vi "Load_ESR.vi"(8 "Tset setting":dbl=800.0, 9 "N per point":i32=7, 10 "wait time adjustment (":dbl, 11 "wait time adjustment":dbl) -> (0 "Unaveraged data":string[][](array[string]), 1 "Array":string[][](array[string]), 2 "Data":string[][](array[string]))   [LabVIEW 2025]
uses:
  MW_resource_name.vi
panel:
  out "error out 3":errorcluster
  out "reference out":refnum<k15>
  in  "RF:Power Level (dBm)":dbl
  in  "Invert pass?":bool=TRUE
  out "Passes":i32
  in  "How many passes?":i32=3
  out "Total Points":dbl
  in  "Step Size":string=".25"
  in  "Ending Frequency":string="3100"
  in  "Starting frequency":string="2650"
  # "A gate delay Typically at 1.25 us\nwidth 300 ns"
  # "18.5 Max"
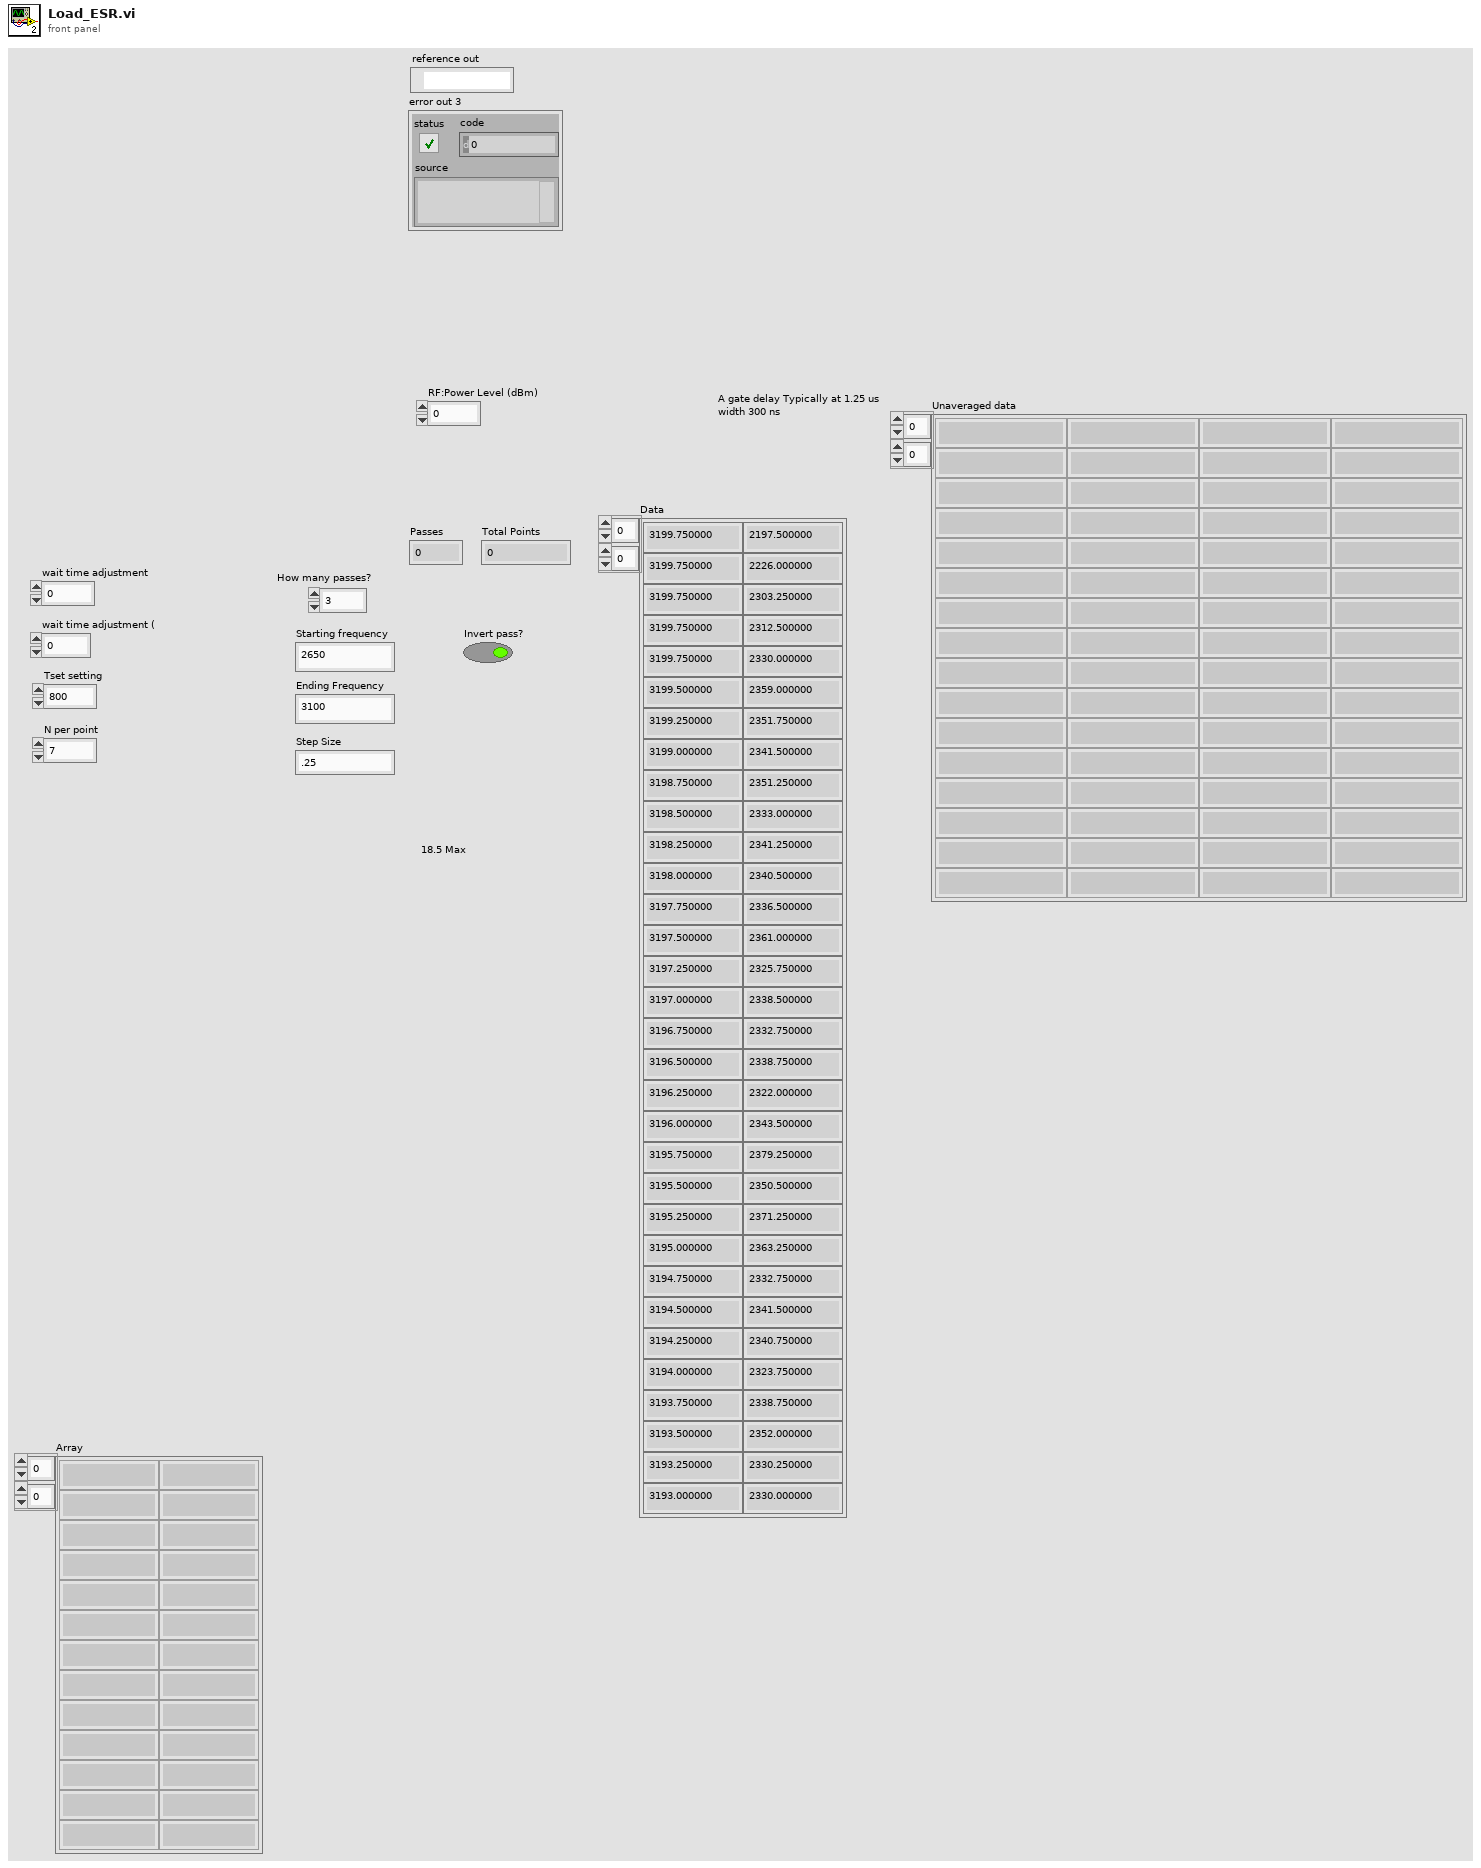
[diagram p1: front panel]
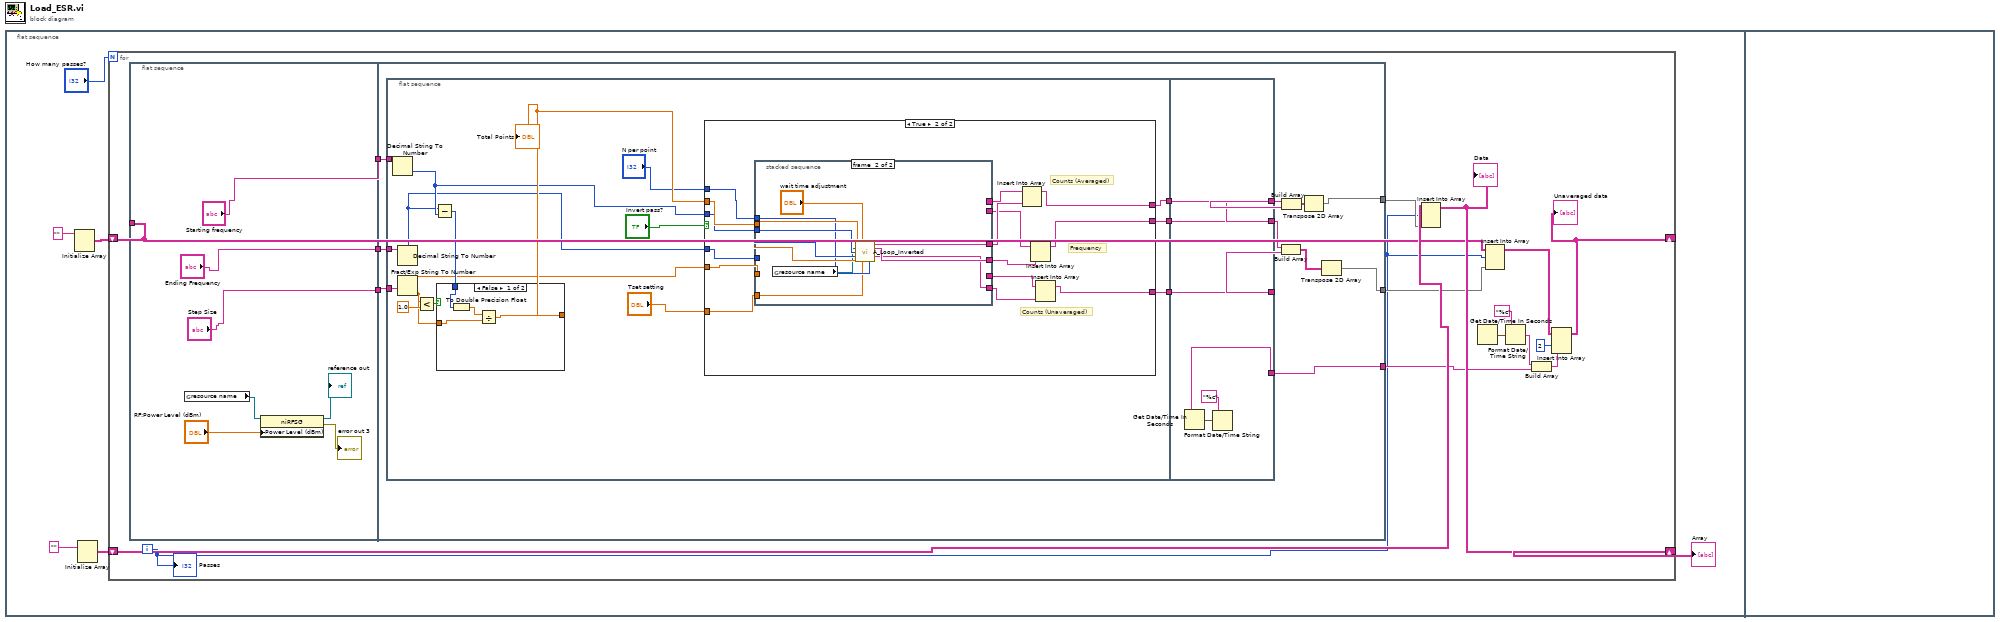
[diagram p0: block diagram]
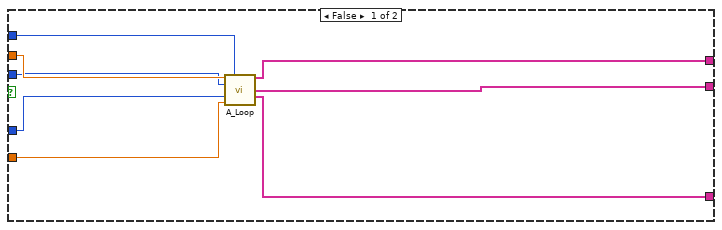
[diagram p2: hidden frame]
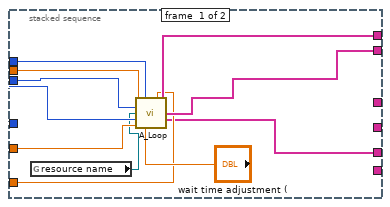
[diagram p3: hidden frame]
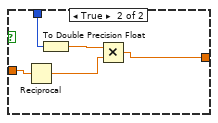
[diagram p4: hidden frame]
diagram:
  n1 = flat-sequence {
    frame #0 {
      n2 = Initialize Array("") -> (w1:string[][])  [unwired: 2 in]
      n3 = Initialize Array("") -> (w4:string[][])  [unwired: 2 in]
      n4 = for {
        N: "How many passes?" -> [_]
        shift-right: [w19] -> w3
        shift-left: w4 -> [w20]
        shift-right: [w12] -> _
        shift-left: w1 -> [w11]
        i -> [w7]
        n5 = flat-sequence {
          tunnel: ["Starting frequency"] -> w23
          tunnel: ["Ending Frequency"] -> w22
          tunnel: ["Step Size"] -> w21
          tunnel: w11 -> [_]
          tunnel: w23 -> [w44]
          tunnel: w22 -> [w43]
          tunnel: w21 -> [w42]
          tunnel: [w40] -> w9
          tunnel: [w38] -> w18
          tunnel: [w31] -> w8
          frame #0 {
            n6 = global read "MW_resource_name.vi" "resource name"() -> (w24:refnum<k15>)
            n7 = property class="niRFSG"(reference=w24, "Power Level (dBm)"="RF:Power Level (dBm)") -> (reference out=→"reference out":refnum<k15>, error out=→"error out 3":errorcluster)  [unwired: 1 in]
          }
          frame #1 {
            n8 = flat-sequence {
              tunnel: w44 -> [w60]
              tunnel: w43 -> [w59]
              tunnel: w42 -> [w57]
              tunnel: [w45] -> w34
              tunnel: [w47] -> w33
              tunnel: [w46] -> w32
              tunnel: [w118] -> w36
              tunnel: [w119] -> w37
              tunnel: [w120] -> w39
              tunnel: w34 -> [w120]
              tunnel: w33 -> [w119]
              tunnel: w32 -> [w118]
              tunnel: [w115] -> w31
              frame #0 {
                n9 = Decimal String To Number(string=w60) -> (number=w52:i32)  [unwired: 2 in, 1 out]
                n10 = Decimal String To Number(string=w59) -> (number=w51:i32)  [unwired: 2 in, 1 out]
                n11 = Fract/Exp String To Number(string=w57) -> (number=w50:dbl)  [unwired: 3 in, 1 out]
                n12 = Less?(x=w50, y=1.0) -> (x < y?=w58:bool)
                n13 = Subtract(x=w51, y=w52) -> (x-y=w55:i32)
                n14 = case shown="False" w58 {
                  tunnel: w50 -> [w107 w114]
                  tunnel: w55 -> [w109 w112]
                  tunnel: [w106 w110] -> w53
                  frame False {
                    n15 = To Double Precision Float(number=w109) -> (double precision float=w108:dbl)
                    n16 = Divide(x=w108, y=w107) -> (x/y=w106:dbl)
                  }
                  frame True {
                    n17 = Reciprocal(x=w114) -> (1/x=w111:dbl)
                    n18 = To Double Precision Float(number=w112) -> (double precision float=w113:dbl)
                    n19 = Multiply(x=w113, y=w111) -> (x*y=w110:dbl)
                  }
                }
                "Total Points" <- w53
                n20 = case shown="True" "Invert pass?" {
                  tunnel: w53 -> [w68 w83]
                  tunnel: w52 -> [w67 w82]
                  tunnel: w51 -> [w66 w81]
                  tunnel: w50 -> [w65 w80]
                  tunnel: [w64 w69] -> w45
                  tunnel: [w63 w70] -> w47
                  tunnel: "N per point" -> [w62 w77]
                  tunnel: "Tset setting" -> [_ w76]
                  tunnel: [w61 w71] -> w46
                  frame False {
                    n21 = call "A_Loop.vi"("Numeric"=w68, "N per point"=w62, "Numeric 2"=w67, "Numeric 3"=w66, "Numeric 4"=w65) -> ("Averaged"=w64:string[], "Frequency"=w63:string[], "Unaveraged"=w61:string[])  [unwired: 6 in, 2 out]
                  }
                  frame True {
                    # "Counts (Unaveraged)"
                    # "Counts (Averaged)"
                    # "Frequency"
                    n22 = stacked-sequence {
                      tunnel: w83 -> [w92 w100]
                      tunnel: w82 -> [w91 w101]
                      tunnel: w81 -> [w90 w103]
                      tunnel: w80 -> [w89 w102]
                      tunnel: [_ w105] -> w75
                      tunnel: [_ w104] -> w78
                      tunnel: [w94 _] -> w79
                      tunnel: [w93 _] -> w73
                      tunnel: w77 -> [w87 w98]
                      tunnel: w76 -> [w86 w97]
                      tunnel: [_ w96] -> w72
                      tunnel: [w85 _] -> w74
                      frame #0 {
                        n23 = global read "MW_resource_name.vi" "resource name"() -> (w84:refnum<k15>)
                        n24 = call "A_Loop.vi"("Numeric"=w92, "N per point"=w87, "Tset setting"=w86, "Numeric 2"=w91, "instrument handle out"=w84, "Numeric 3"=w90, "Numeric 4"=w89, "x"="wait time adjustment (") -> ("Averaged"=w94:string[], "Frequency"=w93:string[], "Unaveraged"=w85:string[])  [unwired: 3 in, 2 out]
                      }
                      frame #1 {
                        n25 = global read "MW_resource_name.vi" "resource name"() -> (w95:refnum<k15>)
                        n26 = call "A_Loop_Inverted.vi"("Numeric"=w100, "x"="wait time adjustment", "instrument handle out"=w95, "Numeric 2"=w101, "Numeric 3"=w103, "Numeric 4"=w102, "Tset setting"=w97, "N per point"=w98) -> ("output array"=w105:string[], "output array 2"=w104:string[], "Array 3"=w96:string[])  [unwired: 5 in]
                      }
                    }
                    n27 = Insert Into Array(array=w79, new element=w75) -> (w69:string[])  [unwired: 1 in]
                    n28 = Insert Into Array "Insert Into Array"(array=w73, new element=w78) -> (w70:string[])  [unwired: 1 in]
                    n29 = Insert Into Array "Insert Into Array"(array=w74, new element=w72) -> (w71:string[])  [unwired: 1 in]
                  }
                }
              }
              frame #1 {
                n30 = Get Date/Time In Seconds() -> (seconds since 1Jan1904=w116:timestamp)
                n31 = Format Date/Time String(time format string (%c)="%c", seconds (now)=w116) -> (date/time string=w115:string)  [unwired: 1 in]
              }
            }
            n32 = Build Array(w37, w36) -> (w35:string[][])
            n33 = Build Array(w37, w39) -> (w41:string[][])
            n34 = Transpose 2D Array(2D array=w41) -> (transposed array=w40:string[][])
            n35 = Transpose 2D Array(2D array=w35) -> (transposed array=w38:string[][])
          }
        }
        n36 = Insert Into Array(array=w20, index (row)=w7, new element=w9) -> (w19:string[][])  [unwired: 1 in]
        "Data" <- w19
        n37 = Get Date/Time In Seconds() -> (seconds since 1Jan1904=w17:timestamp)
        n38 = Insert Into Array(array=w11, index (row)=w7, new element=w18) -> (w10:string[][])  [unwired: 1 in]
        n39 = Format Date/Time String(time format string (%c)="%c", seconds (now)=w17) -> (date/time string=w16:string)  [unwired: 1 in]
        n40 = Build Array(w16, w8) -> (w15:string[])
        n41 = Insert Into Array "Insert Into Array"(array=w10, index (col)=2 ("disabled index (col)"), new element=w15) -> (w12:string[][])  [unwired: 1 in]
        "Unaveraged data" <- w12
        "Passes" <- w7
      }
      "Array" <- w3
    }
    frame #1 {
    }
  }
